vi "ZM-PC-getHeader.vi"(8 "error in (no error)":errorcluster, 11 "ZM-PC-package in":refnum<class "ZM-PC-package.lvclass">) -> (0 "error out":errorcluster, 2 "header":T1, 3 "ZM-PC-package out":refnum<class "ZM-PC-package.lvclass">)   [LabVIEW 2020, in "ZM-PC-packages.lvlib" / "ZM-PC-package.lvclass"]
doc: "Returns the package header as the ZM-PC-HEADER cluster {timestamp, type, destination} of strings, bundled from getTimestampString, getTypeName and getDestinationName. Protected: used by every getDataAsJson."
uses:
  ZM-PC-package.lvclass
  ZM-PC-HEADER.ctl
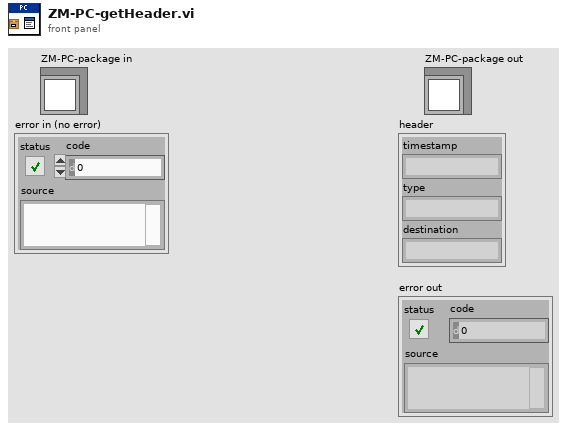
[diagram p1: front panel]
types:
  T1 = typedef "ZM-PC-packages.lvlib/ZM-PC-package.lvclass/ZM-PC-HEADER.ctl" = cluster{"timestamp":string, "type":string, "destination":string}
  T2 = cluster{"timestamp":string, "type":string, "destination":string}
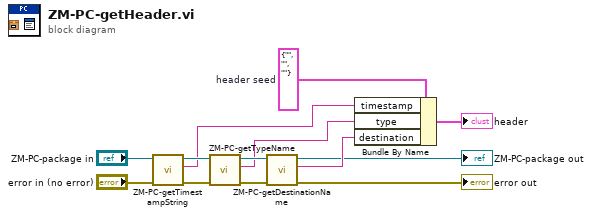
[diagram p0: block diagram]
diagram:
  w4 = T2 {"timestamp"="", "type"="", "destination"=""}  # header seed
  n1 = call "ZM-PC-getTimestampString.vi"("error in (no error)"="error in (no error)", "ZM-PC-package in"="ZM-PC-package in") -> ("error out"=w10:errorcluster, "timestamp_iso"=w7:string, "ZM-PC-package out"=w11:refnum<class "ZM-PC-package.lvclass">)  [unwired: 7 in]
  n2 = call "ZM-PC-getTypeName.vi"("error in (no error)"=w10, "ZM-PC-package in"=w11) -> ("error out"=w8:errorcluster, "type_name"=w6:string, "ZM-PC-package out"=w9:refnum<class "ZM-PC-package.lvclass">)  [unwired: 7 in]
  n3 = call "ZM-PC-getDestinationName.vi"("error in (no error)"=w8, "ZM-PC-package in"=w9) -> ("error out"=→"error out":errorcluster, "destination_name"=w5:string, "ZM-PC-package out"=→"ZM-PC-package out":refnum<class "ZM-PC-package.lvclass">)  [unwired: 7 in]
  n4 = Bundle By Name(cluster=w4, "timestamp"=w7, "type"=w6, "destination"=w5) -> (→"header":T2)
